vi "CreateTemplateChildCfg.vi"(8 "error in (no error)":errorcluster, 9 "Data":T1, 10 "Name":string, 11 "object in":refnum<class "Template_CFG.lvclass">) -> (0 "error out":errorcluster, 3 "object out":refnum<class "Template_CFG.lvclass">)   [LabVIEW 2021, in "Template-Channels.lvlib" / "Template_CFG.lvclass"]
uses:
  Template_CFG.lvclass
  C:/Users/averna/Documents/LV Gym DEMO/Factory Pattern/Generic Channel/Configuration/Configuration.lvclass
  tdef/Data.ctl
  Template_CFG.lvclass/Template_CFG.ctl
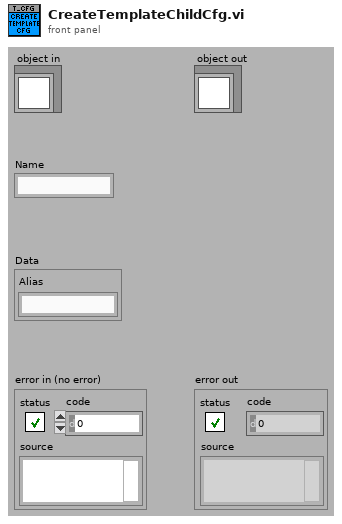
[diagram p1: front panel]
types:
  T1 = typedef "Template-Channels.lvlib/Template_CFG.lvclass/Data.ctl" = cluster{"Alias":string}
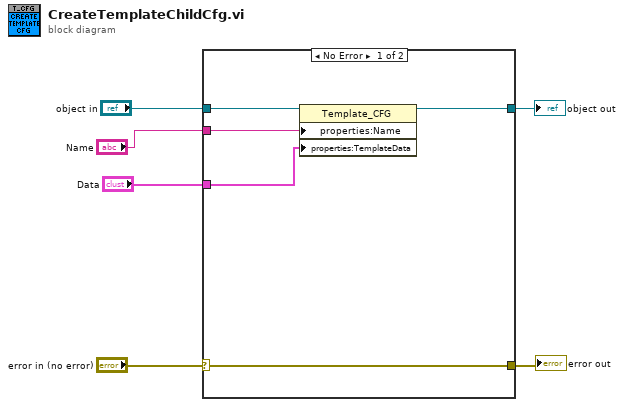
[diagram p0: block diagram]
diagram:
  n1 = case shown="No Error" "error in (no error)" {
    selector: "error in (no error)" -> [w11 w13]
    tunnel: [w11 w13] -> w5
    tunnel: [w9 w12] -> w3
    tunnel: "object in" -> [w10 w12]
    tunnel: "Name" -> [w8 _]
    tunnel: "Data" -> [w7 _]
    frame No Error {
      n2 = property class="Template_CFG"(reference=w10, "properties:Name"=w8, "properties:TemplateData"=w7) -> (reference out=w9:refnum<class "Template_CFG.lvclass">)  [unwired: 1 in, 1 out]
    }
    frame Error {
    }
  }
  "error out" <- w5
  "object out" <- w3
